vi "three_pitcher.vi"() -> ()   [LabVIEW 2021]
panel:
  out "result path":i32[][](array[numeric])
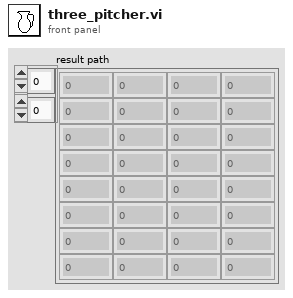
[diagram p1: front panel]
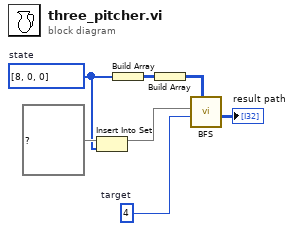
[diagram p0: block diagram]
diagram:
  w2 = 4  # target
  w5 = i32[] [8, 0, 0]  # state
  n1 = Insert Into Set(10:w5, 11:set{i32[]} {} ("set in")) -> (3:w3:set{i32[]})  [unwired: 1 out]
  n2 = Build Array(w5) -> (w1:i32[][])
  n3 = Build Array(w1) -> (w4:i32[][][])
  n4 = call "BFS.vi"("paths"=w4, "target"=w2, "processed states"=w3) -> ("result path"=→"result path":i32[][])  [unwired: 8 in]
